vi "Test MQTT-3.2.0-1.vi"(8 "error in (no error)":errorcluster, 11 "Connection Config":refnum<class "Connection.lvclass">) -> (0 "error out":errorcluster, 3 "Connection Config dup":refnum<class "Connection.lvclass">)   [LabVIEW 2013]
uses:
  <vilib>/LabVIEW Open Source Project/MQTT Control Packets/Control Packets/CONNECT/CONNECT.lvclass
  <vilib>/LabVIEW Open Source Project/MQTT Control Packets/Control Packets/ControlPacket/ControlPacket.lvclass
  <vilib>/addons/_JKI Toolkits/Caraya/classes/Test/Test.lvclass
  <vilib>/addons/_JKI Toolkits/Caraya/classes/Assert/Assert.lvclass
  <vilib>/LabVIEW Open Source Project/MQTT Control Packets/Control Packets/DISCONNECT/DISCONNECT.lvclass
  <vilib>/LabVIEW Open Source Project/MQTT Control Packets/Control Packets/CONNACK/CONNACK.lvclass
  <vilib>/LabVIEW Open Source Project/MQTT Control Packets/Control Packets/CONNACK/Connect Return Code -- enum.ctl
  <vilib>/LabVIEW Open Source Project/Connection/Connection/Connection.lvclass
  <vilib>/LabVIEW Open Source Project/MQTT Connection/MQTT_Connection/Connection/Connection.lvclass
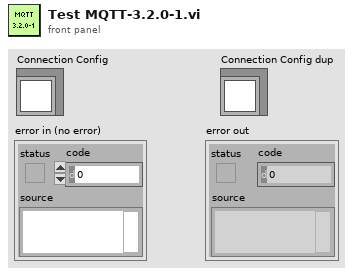
[diagram p1: front panel]
types:
  T1 = enum16{"Standard", "Buffered", "CRLF", "Immediate"}
  T2 = typedef "MQTT_Control_Packets.lvlib/CONNACK.lvclass/Connect Return Code -- enum.ctl" = enum16{"Connection accepted", "Unacceptable protocol version", "Identifier Rejected", "Server Unavailable", "Bad Username or Password", "Not Authorized"}
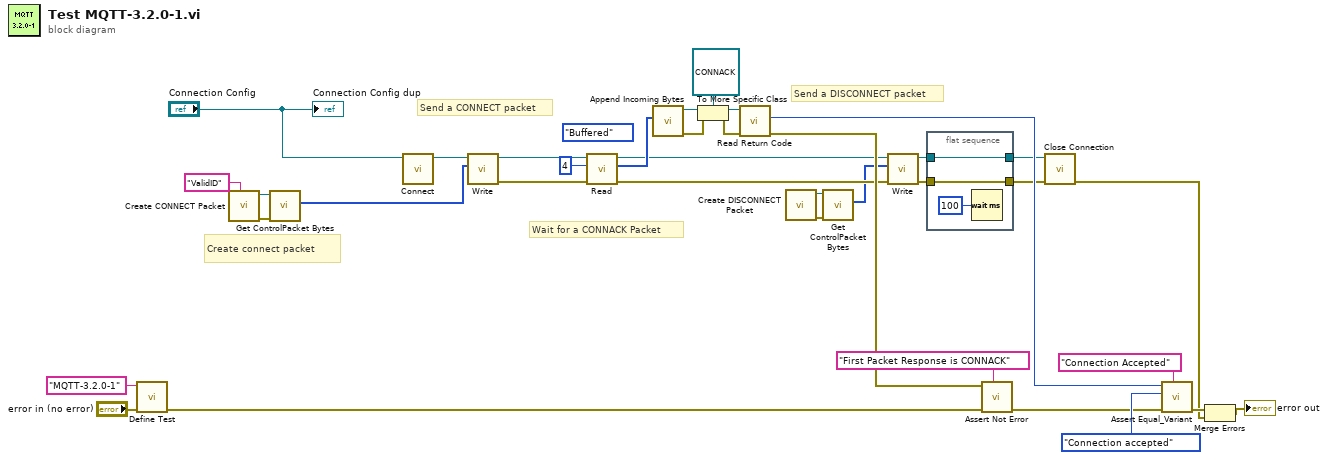
[diagram p0: block diagram]
diagram:
  (unwired) T1."Buffered" ("mode (standard)")
  # "Send a DISCONNECT packet"
  # "Wait for a CONNACK Packet"
  # "Create connect packet"
  # "Send a CONNECT packet"
  n1 = call <vilib>:"Define Test.vi"("error in (no error)"="error in (no error)", "Label (VI Title)"="MQTT-3.2.0-1") -> ("error out"=w17:errorcluster)  [unwired: 9 in]
  n2 = call <vilib>:"Create CONNECT Packet.vi"("Client ID (empty: generate new)"="ValidID") -> ("error out"=w35:errorcluster, "CONNECT"=w36:refnum<class "CONNECT.lvclass">)  [unwired: 8 in, 1 out]
  n3 = call <vilib>:"Get ControlPacket Bytes.vi"("error in (no error)"=w35, "ControlPacket"=w36) -> ("Bytes Stream"=w15:u8[])  [unwired: 6 in, 3 out]
  n4 = call <vilib>:"Connect.vi"("Connection in"="Connection Config") -> ("Connection out"=w2:refnum<class "Connection.lvclass">)  [unwired: 9 in, 1 out]
  n5 = call <vilib>:"Write.vi"("Bytes"=w15, "Connection in"=w2) -> ("error out"=w13:errorcluster, "Connection"=w14:refnum<class "Connection.lvclass">)  [unwired: 8 in]
  n6 = call <vilib>:"Read.vi"("error in (no error)"=w13, "bytes to read (100)"=4 ("bytes to read"), "TCPConnection in"=w14) -> ("error out"=w5:errorcluster, "Bytes"=w11:u8[], "TCPConnection out"=w7:refnum<class "Connection.lvclass">)  [unwired: 4 in, 2 out]
  n7 = call <vilib>:"Append Incoming Bytes.vi"("Incoming Packets"=w11) -> ("error out"=w19:errorcluster, "ControlPacket"=w27:refnum<class "ControlPacket.lvclass">)  [unwired: 7 in, 2 out]
  n8 = To More Specific Class(target class=refnum<class "CONNACK.lvclass"> refnum ("CONNACK in"), reference=w27, error in=w19) -> (specific class reference=w26:refnum<class "CONNACK.lvclass">, error out=w23:errorcluster)
  n9 = call <vilib>:"Read Return Code.vi"("error in (no error)"=w23, "CONNACK in"=w26) -> ("error out"=w21:errorcluster, "Return Code"=w25:T2)  [unwired: 7 in, 1 out]
  n10 = call <vilib>:"Create DISCONNECT Packet.vi"() -> ("error out"=w29:errorcluster, "DISCONNECT"=w28:refnum<class "DISCONNECT.lvclass">)  [unwired: 9 in, 1 out]
  n11 = call <vilib>:"Get ControlPacket Bytes.vi"("error in (no error)"=w29, "ControlPacket"=w28) -> ("Bytes Stream"=w3:u8[])  [unwired: 6 in, 3 out]
  n12 = call <vilib>:"Write.vi"("error in (no error)"=w5, "Bytes"=w3, "Connection in"=w7) -> ("error out"=w4:errorcluster, "Connection"=w6:refnum<class "Connection.lvclass">)  [unwired: 7 in]
  n13 = flat-sequence {
    tunnel: w6 -> [w39]
    tunnel: [w39] -> w10
    tunnel: [w37] -> w9
    tunnel: w4 -> [w37]
    frame #0 {
      n14 = Wait (ms)(milliseconds to wait=u32 100) -> ()  [unwired: 1 out]
    }
  }
  n15 = call <vilib>:"Assert Not Error.vi"("Label"="First Packet Response is CONNACK", "error in (no error)"=w17, "Not Error?"=w21) -> ("error out"=w22:errorcluster)  [unwired: 8 in]
  n16 = call <vilib>:"Close Connection.vi"("error in (no error)"=w9, "Connection in"=w10) -> ("error out"=w8:errorcluster)  [unwired: 8 in, 1 out]
  n17 = call <vilib>:"Assert Equal_Variant.vi"("Label"="Connection Accepted", "error in (no error)"=w22, "Y"=Connect_Return_Code_--_enum."Connection accepted" ("Return Code"), "X"=w25) -> ("error out"=w33:errorcluster)  [unwired: 7 in]
  n18 = Merge Errors(w33, w8) -> (→"error out":errorcluster)
  "Connection Config dup" <- "Connection Config"
